vi "VIH HelpGen - HTML - Extract Template Codes.vi"(9 "Tag names":string[](array[string]), 11 "HTML in":string) -> (1 "Templates":string[](array[string]), 3 "HTML out":string)   [LabVIEW 2014]
doc: "::: VI Helpeks :::\nCopyright (c) 2000-2026 Konstantin Shifershteyn. All rights reserved."
panel:
  # "VI Helpeks\nCopyright (c) 2012-2026 Konstantin Shifershteyn"
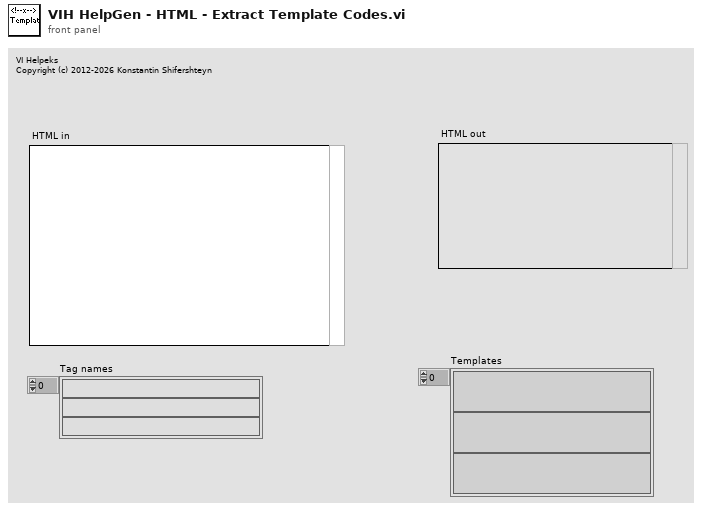
[diagram p1: front panel]
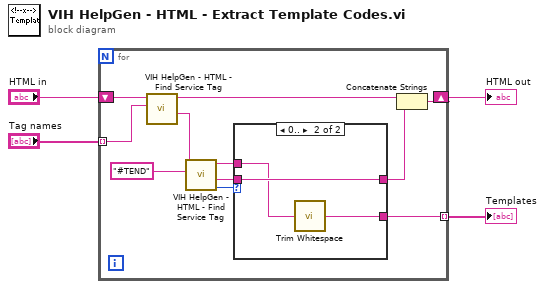
[diagram p0: block diagram]
diagram:
  n1 = for {
    tunnel: "Tag names" -> [w9] mode=indexing
    shift-right: [w15] -> w3
    shift-left: "HTML in" -> [w12]
    tunnel: [w13] -> w1 mode=indexing
    n2 = call "VIH HelpGen - HTML - Find Service Tag.vi"("Tag name"=w9, "HTML in"=w12) -> ("After"=w10:string, "Before"=w11:string)  [unwired: 6 in, 2 out]
    n3 = call "VIH HelpGen - HTML - Find Service Tag.vi"("Tag name"="#TEND", "HTML in"=w10) -> ("Offset out"=w5:i32, "After"=w6:string, "Before"=w8:string)  [unwired: 6 in, 1 out]
    n4 = case shown="0.." w5 {
      tunnel: w6 -> [_ w19]
      tunnel: [w16 w19] -> w14
      tunnel: w8 -> [w16 w18]
      tunnel: [_ w17] -> w13
      frame ..-1 {
      }
      frame 0.. {
        n5 = call <vilib>:"Trim Whitespace.vi"("string"=w18) -> ("trimmed string"=w17:string)  [unwired: 1 in]
      }
    }
    n6 = Concatenate Strings(w11, w14) -> (w15:string)
  }
  "HTML out" <- w3
  "Templates" <- w1
